vi "Read any file waveform.vi"(4 "(BINARY) 2D number of rows":i32, 6 "(BINARY) 2D number of columns/1D count (all as 1D: -1)":i32=1, 7 "tdms file in":refnum<k34>, 8 "error in":errorcluster, 9 "Data File Type":T2(ring), 10 "Data window":T1={"Start"=0, "Length"=500000, "Channel numbers"=[0], "Channel names"=["Bdot", "Freq"], "Group name"="Untitled"}, 11 "Input file path":path) -> (0 "error out":errorcluster, 1 "1st channel length":u64, 2 "Data out":waveform(dbl)[](array[waveform]), 3 "Actual input file path":path, 5 "tdms file out":refnum<k34>)   [LabVIEW 2018]
panel:
  out "Header":string
  # "OR"
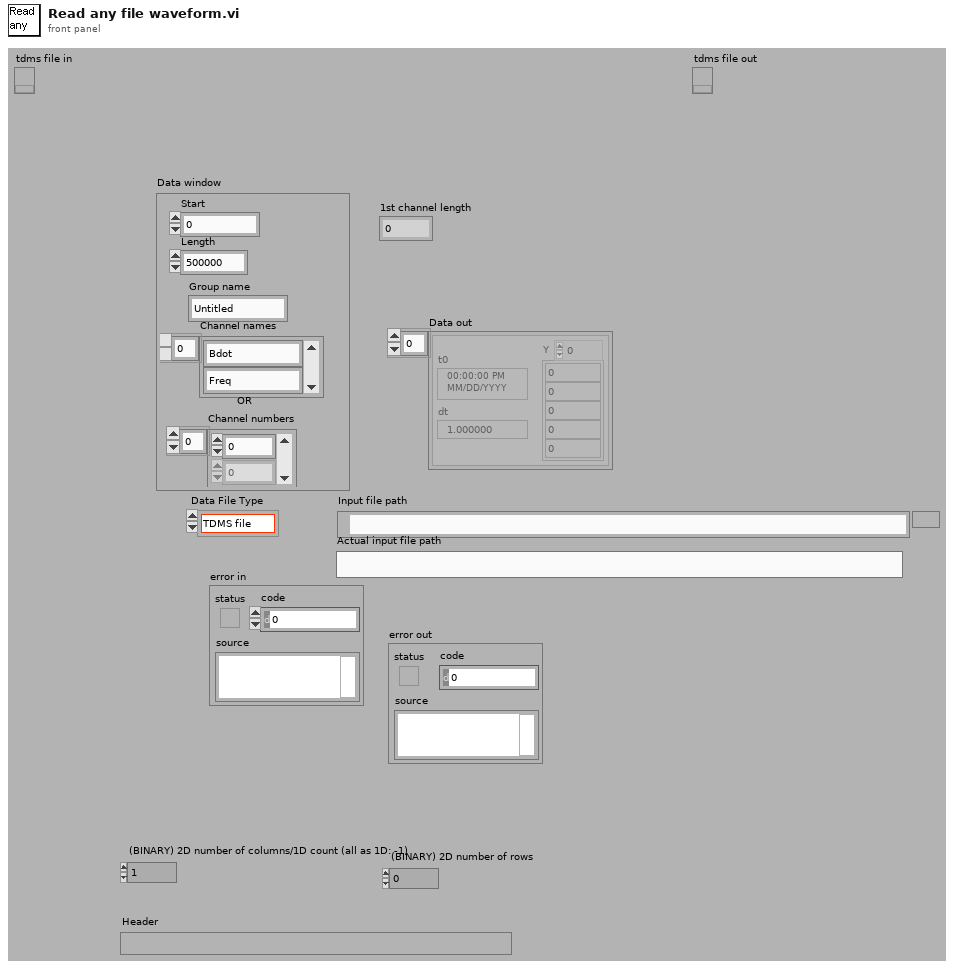
[diagram p1: front panel]
types:
  T1 = cluster{"Start":i64, "Length":i64, "Channel numbers":i64[], "Channel names":string[], "Group name":string}
  T2 = enum16{"TDMS file", "Tektronics ISF", "BinF file", "ASCII File", "BinH File", "BinW File", "BINARY File"}
  T3 = enum16{"open", "open or create", "create or replace", "create", "open (read-only)"}
  T4 = cluster{"Version":i16, "Data Representation":enum16{"Undefined", "I8", "I16", "I32", "I64", "U8", "U16", "U32", "U64", "SGL", "DBL", "EXT"}, "# columns (samples per channel)":i64, "# rows (channels)":i64, "# pre-trigger samples":i64, "Sample rate":dbl, "ADC offset":dbl, "Scale factor":dbl}
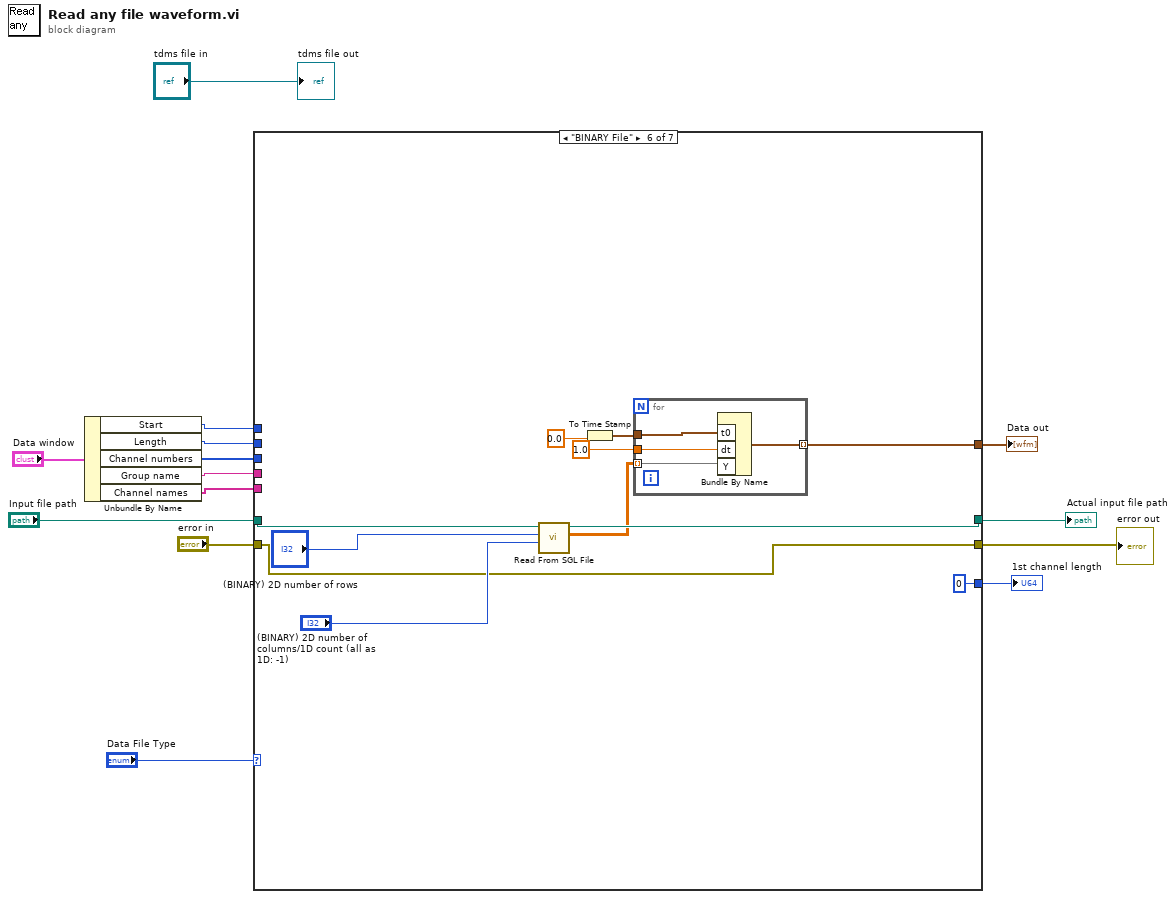
[diagram p0: block diagram]
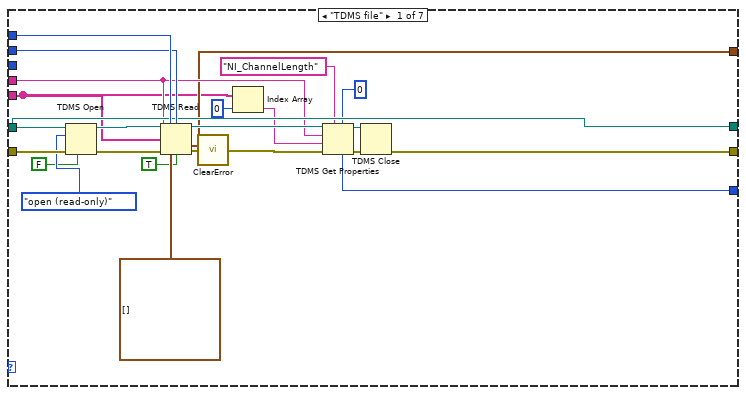
[diagram p2: hidden frame]
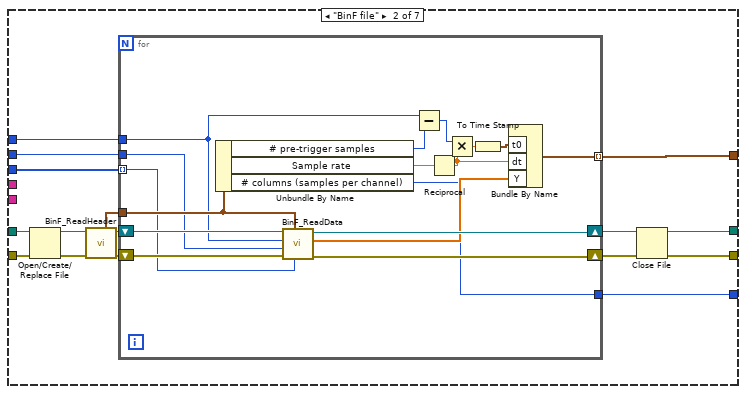
[diagram p3: hidden frame]
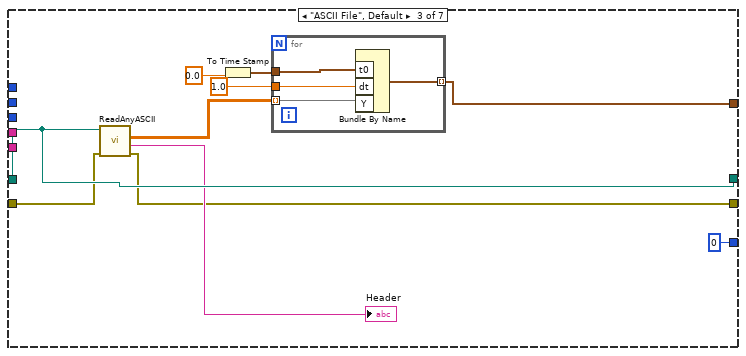
[diagram p4: hidden frame]
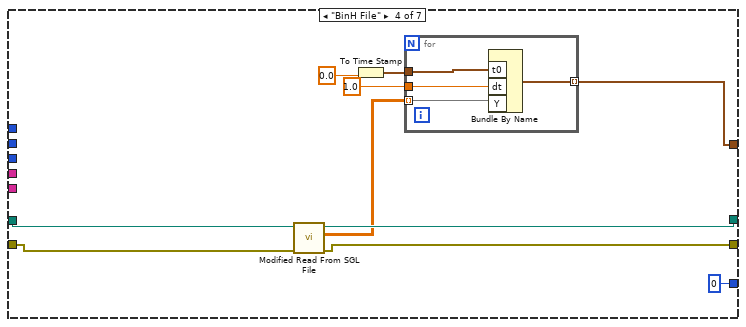
[diagram p5: hidden frame]
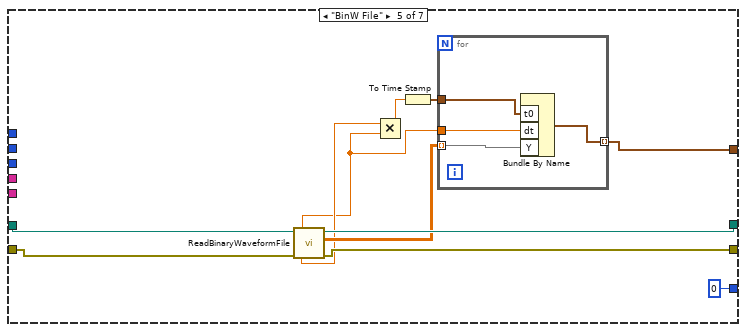
[diagram p6: hidden frame]
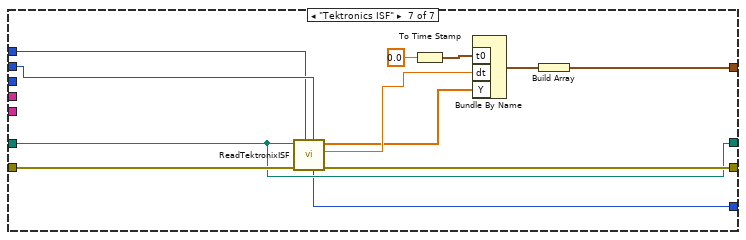
[diagram p7: hidden frame]
diagram:
  n1 = Unbundle By Name("Data window") -> ("Start"=w9:i64, "Length"=w8:i64, "Channel numbers"=w10:i64[], "Group name"=w4:string, "Channel names"=w6:string[])
  n2 = case shown="\"BINARY File\"" "Data File Type" {
    tunnel: "Input file path" -> [w31 w52 w75 w95 w110 w125 w132]
    tunnel: [w31 w44 w75 w94 w109 w124 w132] -> w12
    tunnel: "error in" -> [w38 w51 w73 w93 w108 w117 w135]
    tunnel: [w19 w45 w72 w92 w107 w117 w134] -> w2
    tunnel: w10 -> [_ w43 _ _ _ _ _]
    tunnel: w9 -> [w34 w42 _ _ _ _ w136]
    tunnel: w8 -> [w33 w41 _ _ _ _ w137]
    tunnel: [w21 w40 w78 w88 w106 w121 w131] -> w7
    tunnel: w6 -> [w18 _ _ _ _ _ _]
    tunnel: [w23 w39 u64 0 ("# columns (samples per channel)") u64 0 ("# columns (samples per channel)") u64 0 ("# columns (samples per channel)") u64 0 ("# columns (samples per channel)") w130] -> w5
    tunnel: w4 -> [w22 _ _ _ _ _ _]
    frame "TDMS file" {
      n3 = TDMS Open(6:FALSE ("disable buffering (T)"), 8:w38, 10:T3."open (read-only)" ("operation (0:open)"), 11:w31) -> (0:w36:errorcluster, 3:w37:refnum<k34>)  [unwired: 3 in]
      n4 = TDMS Read(0:w37, 1:w34, 2:w33, 5:w22, 7:w18, 11:w36, 12:waveform(dbl)[] [], 13:TRUE ("return channels in file order? (F)")) -> (4:w29:refnum<k34>, 10:w21:waveform(dbl)[], 15:w17:errorcluster)  [unwired: 3 out]
      n5 = call <vilib>:"ClearError.vi"("error in (no error)"=w17) -> ("error out"=w32:errorcluster)
      n6 = Index Array(array=w18, index=0) -> (element=w26:string)
      n7 = TDMS Get Properties(5:u64 0, 7:"NI_ChannelLength" ("property name"), 8:w32, 9:w26, 10:w22, 11:w29) -> (0:w30:errorcluster, 3:w28:refnum<k34>, 4:w23:u64)  [unwired: 3 out]
      n8 = TDMS Close(8:w30, 11:w28) -> (0:w19:errorcluster)  [unwired: 1 out]
    }
    frame "BinF file" {
      n9 = Open/Create/Replace File(file path (use dialog)=w52, error in=w51) -> (refnum out=w53:refnum<file>, error out=w54:errorcluster)  [unwired: 5 out]
      n10 = call "BinF_ReadHeader.vi"("error in"=w54, "refnum"=w53) -> ("error out"=w50:errorcluster, "refnum out"=w49:refnum<file>, "BinF File Settings"=w48:T4)  [unwired: 7 out]
      n11 = for {
        shift-right: [w70] -> w47
        shift-left: w50 -> [w71]
        shift-right: [w68] -> w46
        shift-left: w49 -> [w69]
        tunnel: w48 -> [w61]
        tunnel: w43 -> [w60] mode=indexing
        tunnel: w42 -> [w58]
        tunnel: w41 -> [w59]
        tunnel: [w56] -> w40 mode=indexing
        tunnel: [w55] -> w39
        n12 = Unbundle By Name(w61) -> ("# pre-trigger samples"=w65:i64, "Sample rate"=w63:dbl, "# columns (samples per channel)"=w55:i64)
        n13 = call "BinF_ReadData.vi"("Channel number"=w60, "BinF File Settings"=w61, "error in"=w71, "Length"=w59, "Start"=w58, "refnum"=w69) -> ("error out"=w70:errorcluster, "Channel Data"=w57:sgl[], "refnum out"=w68:refnum<file>)  [unwired: 3 out]
        n14 = Subtract(x=w58, y=w65) -> (x-y=w66:i64)
        n15 = Reciprocal(x=w63) -> (1/x=w64:dbl)
        n16 = Multiply(x=w66, y=w64) -> (x*y=w67:dbl)
        n17 = To Time Stamp(1:w67) -> (0:w62:timestamp)
        n18 = Bundle By Name("t0"=w62, "dt"=w64, "Y"=w57) -> (w56:waveform(sgl))  [unwired: 1 out]
      }
      n19 = Close File(refnum=w46, error in=w47) -> (path=w44:path, error out=w45:errorcluster)
    }
    frame "ASCII File", Default {
      n20 = call "ReadAnyASCII.vi"("error in (no error)"=w73, "file path (dialog if empty)"=w75) -> ("error out"=w72:errorcluster, "Header text"=→"Header":string, "all rows"=w77:dbl[][])  [unwired: 2 in, 5 out]
      n21 = To Time Stamp(1:0.0) -> (0:w80:timestamp)
      n22 = for {
        tunnel: w77 -> [w85] mode=indexing
        tunnel: [w84] -> w78 mode=indexing
        tunnel: w80 -> [w83]
        tunnel: 1.0 -> [w82]
        n23 = Bundle By Name("t0"=w83, "dt"=w82, "Y"=w85) -> (w84:waveform(dbl))  [unwired: 1 out]
      }
    }
    frame "BinH File" {
      n24 = call "Modified Read From SGL File.vi"("error in (no error)"=w93, "file path (dialog if empty)"=w95) -> ("error out"=w92:errorcluster, "2D array"=w87:sgl[][], "new file path (Not A Path if cancelled)"=w94:path)  [unwired: 1 in, 6 out]
      n25 = To Time Stamp(1:0.0) -> (0:w90:timestamp)
      n26 = for {
        tunnel: w87 -> [w99] mode=indexing
        tunnel: [w98] -> w88 mode=indexing
        tunnel: w90 -> [w97]
        tunnel: 1.0 -> [w96]
        n27 = Bundle By Name("t0"=w97, "dt"=w96, "Y"=w99) -> (w98:waveform(sgl))  [unwired: 1 out]
      }
    }
    frame "BinW File" {
      n28 = call "ReadBinaryWaveformFile.vi"("error in (no error)"=w108, "file path (dialog if empty)"=w110) -> ("error out"=w107:errorcluster, "2D array"=w105:sgl[][], "new file path (Not A Path if cancelled)"=w109:path, "Time base"=w104:dbl, "Delay, points"=w101:dbl)  [unwired: 1 in, 4 out]
      n29 = Multiply(x=w104, y=w101) -> (x*y=w103:dbl)
      n30 = To Time Stamp(1:w103) -> (0:w102:timestamp)
      n31 = for {
        tunnel: w105 -> [w113] mode=indexing
        tunnel: [w114] -> w106 mode=indexing
        tunnel: w102 -> [w112]
        tunnel: w101 -> [w111]
        n32 = Bundle By Name("t0"=w112, "dt"=w111, "Y"=w113) -> (w114:waveform(sgl))  [unwired: 1 out]
      }
    }
    frame "BINARY File" {
      n33 = call <vilib>:"Read From SGL File.vi"("2D number of columns/1D count (all as 1D: -1)"="(BINARY) 2D number of columns/1D count (all as 1D: -1)", "2D number of rows"="(BINARY) 2D number of rows", "file path (dialog if empty)"=w125) -> ("2D array"=w122:sgl[][], "new file path (Not A Path if cancelled)"=w124:path)  [unwired: 7 out]
      n34 = To Time Stamp(1:0.0) -> (0:w119:timestamp)
      n35 = for {
        tunnel: w122 -> [w129] mode=indexing
        tunnel: [w128] -> w121 mode=indexing
        tunnel: w119 -> [w127]
        tunnel: 1.0 -> [w126]
        n36 = Bundle By Name("t0"=w127, "dt"=w126, "Y"=w129) -> (w128:waveform(sgl))  [unwired: 1 out]
      }
    }
    frame "Tektronics ISF" {
      n37 = call "ReadTektronixISF.vi"("Length"=w137, "Start"=w136, "error in (no error)"=w135, "Path"=w132) -> ("error out"=w134:errorcluster, "dt"=w141:dbl, "Data"=w133:dbl[], "Total number of points"=w130:u64)  [unwired: 4 out]
      n38 = To Time Stamp(1:0.0) -> (0:w138:timestamp)
      n39 = Bundle By Name("t0"=w138, "dt"=w141, "Y"=w133) -> (w140:waveform(dbl))  [unwired: 1 out]
      n40 = Build Array(w140) -> (w131:waveform(dbl)[])
    }
  }
  "Actual input file path" <- w12
  "error out" <- w2
  "Data out" <- w7
  "1st channel length" <- w5
  "tdms file out" <- "tdms file in"
